vi "G-del_tab.vi"(10 "字符串":string) -> (2 "数组":string[](array[string]))   [LabVIEW 2025, in "G-Uart-Class.lvclass"]
uses:
  G-Uart-Class.lvclass
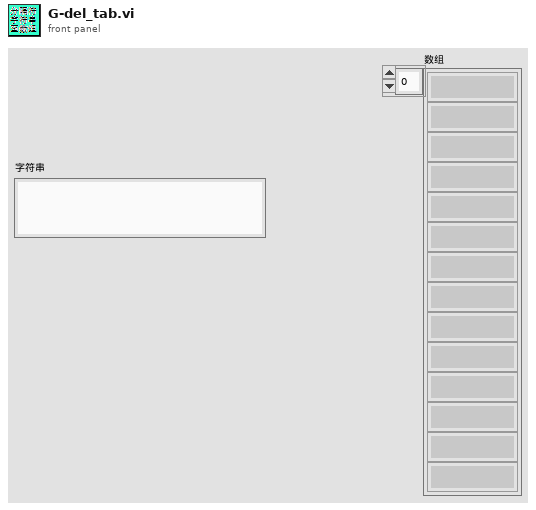
[diagram p1: front panel]
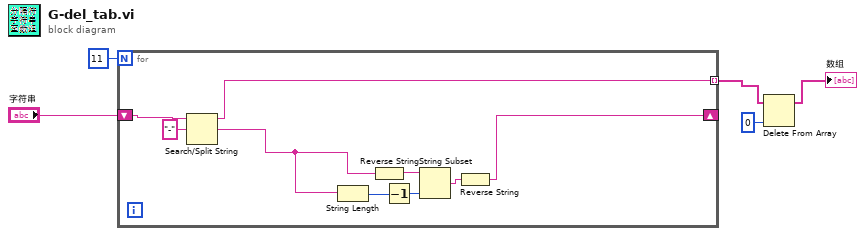
[diagram p0: block diagram]
diagram:
  n1 = for {
    N: 11 -> [_]
    shift-right: [w7] -> _
    shift-left: "字符串" -> [w14]
    tunnel: [w12] -> w3 mode=indexing
    n2 = Search/Split String(string=w14, search string/char (-)="-" ("搜索字符串/字符(-)")) -> (substring before match=w12:string, match + rest of string=w6:string)  [unwired: 1 in, 1 out]
    n3 = String Length(string=w6) -> (length=w10:i32)
    n4 = Reverse String(1:w6) -> (0:w11:string)
    n5 = Decrement(x=w10) -> (x-1=w9:i32)
    n6 = String Subset(string=w11, length (rest)=w9) -> (substring=w8:string)  [unwired: 1 in]
    n7 = Reverse String(1:w8) -> (0:w7:string)
  }
  n8 = Delete From Array(array=w3, index=0 ("索引")) -> (array with subset deleted=→"数组":string[])  [unwired: 1 in, 1 out]
